vi "Assert Less_Variant.vi"(4 "Execution time (s)":dbl=-1.0, 5 "Assert Only? (F)":bool, 6 "error code (1)":i32=1, 7 "Label":string, 8 "error in (no error)":errorcluster, 9 "Register with caller test (F)":bool, 10 "Y":variant, 11 "X":variant) -> (0 "error out":errorcluster, 2 "Properties.Assert":refnum<class "Properties.Assert.lvclass">)   [LabVIEW 2013, in "Caraya.lvlib" / "Assert.lvclass"]
doc: "Generates an error if the input condition is not met.\n\n--\nCopyright © 2015 JKI All rights reserved.\n\nAuthor: Tomi Maila <tomi.maila@jki.net>\n\nThis library is provided \"AS IS\" ,WITHOUT WARRANTIES OR\nCONDITIONS OF ANY KIND, either express or implied.\n\nJKI -- jki.net"
uses:
  Assert.lvclass
  Properties.Assert/Properties.Assert.lvclass
  Properties/Properties.lvclass
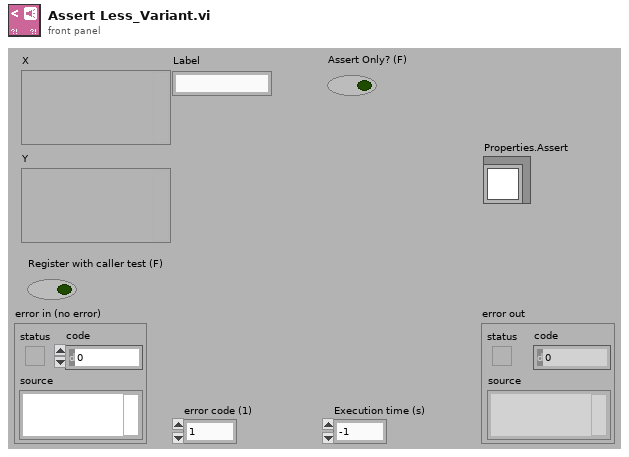
[diagram p1: front panel]
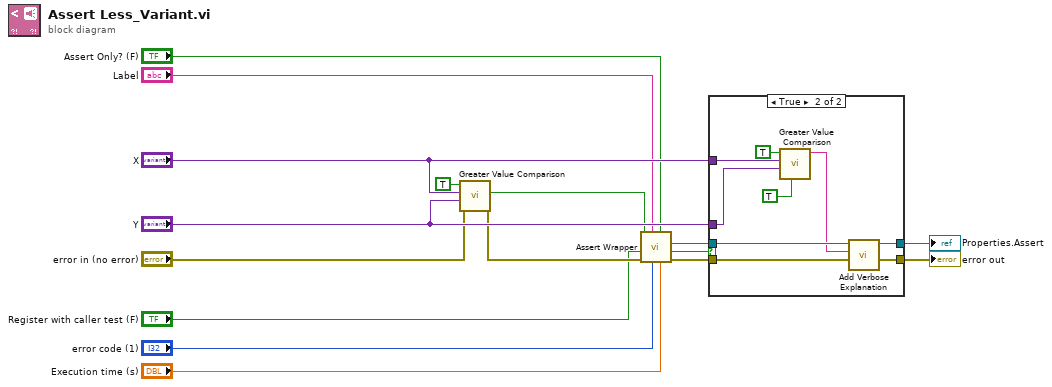
[diagram p0: block diagram]
diagram:
  n1 = call "Greater Value Comparison.vi"("error in (no error)"="error in (no error)", "Y"="Y", "X"="X", "Less Than? (F)"=TRUE) -> ("error out"=w12:errorcluster, "Asserted?"=w11:bool)  [unwired: 5 in, 1 out]
  n2 = call "Assert Wrapper.vi"("Execution time (s)"="Execution time (s)", "Assert Only? (F)"="Assert Only? (F)", "error code (1)"="error code (1)", "Label"="Label", "error in (no error)"=w12, "Register with caller test (F)"="Register with caller test (F)", "Assert?"=w11) -> ("error out"=w16:errorcluster, "Verbose"=w15:bool, "Properties.Assert"=w2:refnum<class "Properties.Assert.lvclass">)  [unwired: 1 in, 1 out]
  n3 = case shown="True" w15 {
    tunnel: [w18 w20] -> w7
    tunnel: w16 -> [w18 w21]
    tunnel: "X" -> [_ w26]
    tunnel: "Y" -> [_ w25]
    tunnel: w2 -> [w17 w23]
    tunnel: [w17 w19] -> w1
    frame False {
    }
    frame True {
      n4 = call "Greater Value Comparison.vi"("verbose? (F)"=TRUE, "Y"=w25, "X"=w26, "Less Than? (F)"=TRUE) -> ("Verbose output"=w22:string)  [unwired: 5 in, 2 out]
      n5 = call "Add Verbose Explanation.vi"("error in (no error)"=w21, "Verbose Explanation"=w22, "Properties"=w23) -> ("error out"=w20:errorcluster, "Properties"=w19:refnum<class "Properties.Assert.lvclass">)  [unwired: 7 in]
    }
  }
  "error out" <- w7
  "Properties.Assert" <- w1
